vi "Host_Params.vi"(4 "Timeout":u16, 5 "Prev Timeout":u16, 6 "Capacity":u16, 7 "Prev Capacity":u16, 8 "Prev Speed":u16, 9 "Speed":u16, 10 "Step":u16, 11 "Queue":refnum<queue>) -> (1 "Next Capacity":u16, 2 "Next Timeout":u16, 3 "Next Speed":u16)   [LabVIEW 2018]
doc: "Use this template to build a VI to use as a subVI."
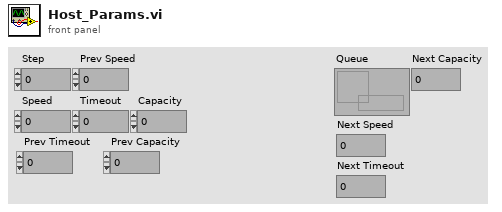
[diagram p1: front panel]
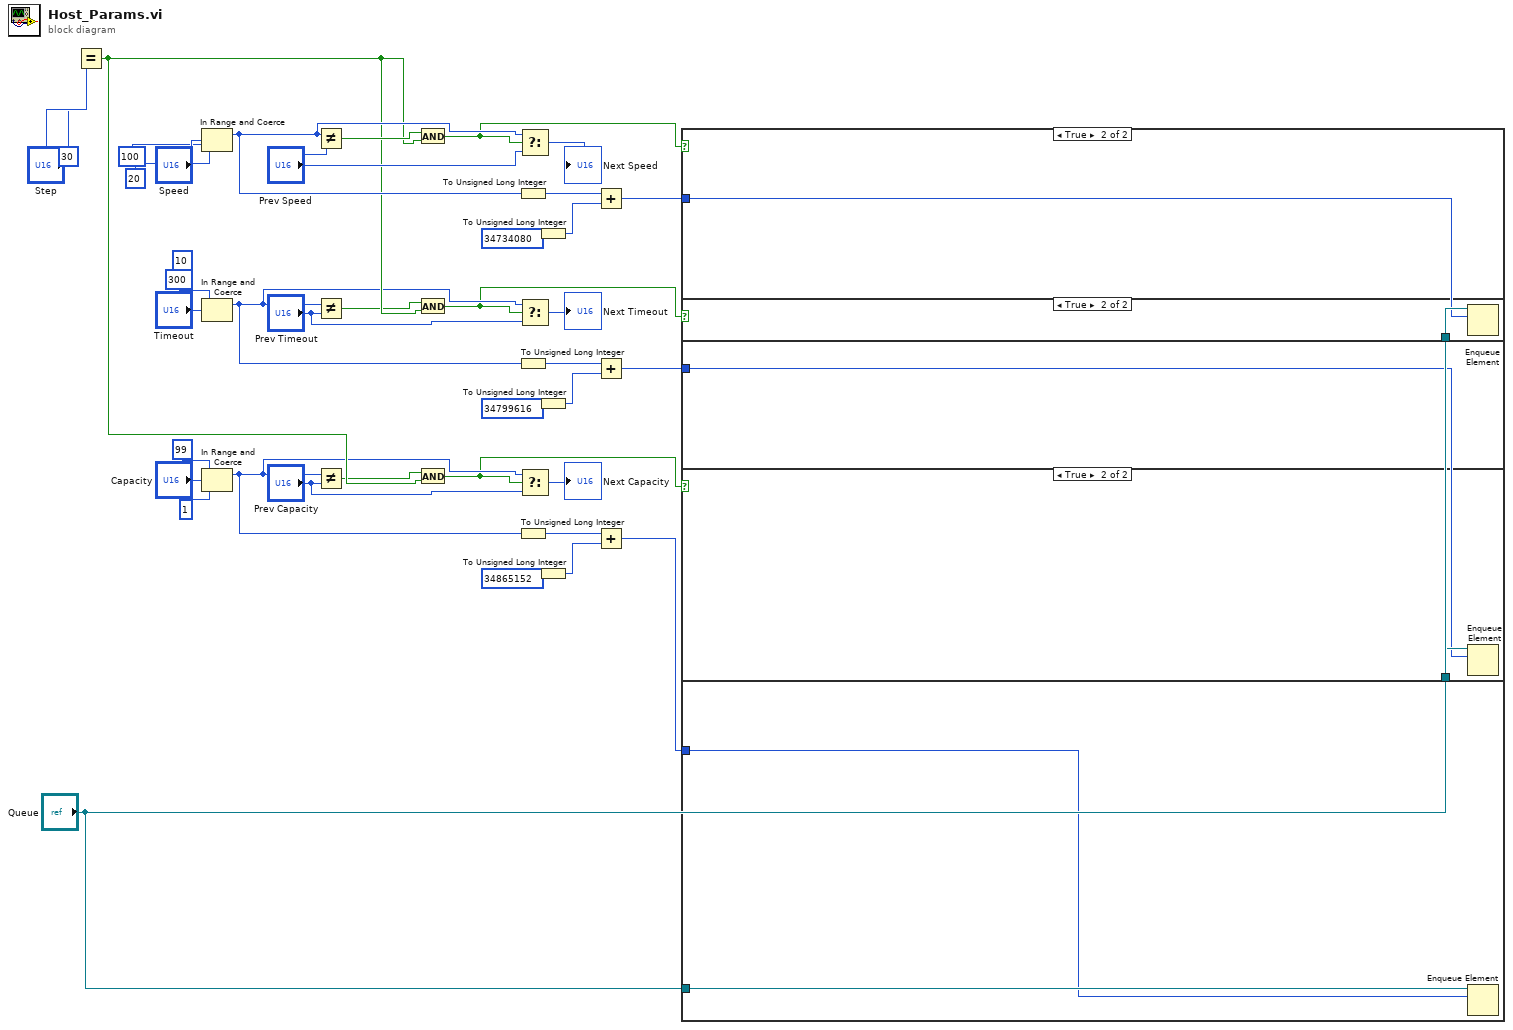
[diagram p0: block diagram]
diagram:
  n1 = Equal?(x="Step", y=u16 30) -> (x = y?=w32:bool)
  n2 = In Range and Coerce(upper limit=u16 100, x="Speed", lower limit=u16 20) -> (coerced(x)=w35:u16)  [unwired: 1 out]
  n3 = In Range and Coerce(upper limit=u16 300, x="Timeout", lower limit=u16 10) -> (coerced(x)=w22:u16)  [unwired: 1 out]
  n4 = In Range and Coerce(upper limit=u16 99, x="Capacity", lower limit=u16 1) -> (coerced(x)=w10:u16)  [unwired: 1 out]
  n5 = Not Equal?(x=w35, y="Prev Speed") -> (x != y?=w33:bool)
  n6 = Not Equal?(x=w22, y="Prev Timeout") -> (x != y?=w20:bool)
  n7 = Not Equal?(x=w10, y="Prev Capacity") -> (x != y?=w8:bool)
  n8 = And(x=w33, y=w32) -> (x .and. y?=w31:bool)
  n9 = And(x=w20, y=w32) -> (x .and. y?=w19:bool)
  n10 = And(x=w8, y=w32) -> (x .and. y?=w7:bool)
  n11 = To Unsigned Long Integer(number=w35) -> (unsigned 32bit integer=w29:u32)
  n12 = To Unsigned Long Integer(number=w22) -> (unsigned 32bit integer=w17:u32)
  n13 = To Unsigned Long Integer(number=w10) -> (unsigned 32bit integer=w5:u32)
  n14 = Select(t=w35, s=w31, f="Prev Speed") -> (s? t:f=→"Next Speed":u16)
  n15 = Select(t=w22, s=w19, f="Prev Timeout") -> (s? t:f=→"Next Timeout":u16)
  n16 = Select(t=w10, s=w7, f="Prev Capacity") -> (s? t:f=→"Next Capacity":u16)
  n17 = To Unsigned Long Integer(number=34734080) -> (unsigned 32bit integer=w27:u32)
  n18 = To Unsigned Long Integer(number=34799616) -> (unsigned 32bit integer=w15:u32)
  n19 = To Unsigned Long Integer(number=34865152) -> (unsigned 32bit integer=w3:u32)
  n20 = Add(x=w29, y=w27) -> (x+y=w26:u32)
  n21 = Add(x=w17, y=w15) -> (x+y=w14:u32)
  n22 = Add(x=w5, y=w3) -> (x+y=w1:u32)
  n23 = case shown="True" w31 {
    tunnel: "Queue" -> [_ w42]
    tunnel: w26 -> [_ w41]
    frame False {
    }
    frame True {
      n24 = Enqueue Element(queue=w42, element=w41) -> ()  [unwired: 2 in, 3 out]
    }
  }
  n25 = case shown="True" w19 {
    tunnel: "Queue" -> [_ w44]
    tunnel: w14 -> [_ w43]
    frame False {
    }
    frame True {
      n26 = Enqueue Element(queue=w44, element=w43) -> ()  [unwired: 2 in, 3 out]
    }
  }
  n27 = case shown="True" w7 {
    tunnel: "Queue" -> [_ w46]
    tunnel: w1 -> [_ w45]
    frame False {
    }
    frame True {
      n28 = Enqueue Element(queue=w46, element=w45) -> ()  [unwired: 2 in, 3 out]
    }
  }
